vi "NEO Set Output.vi"(6 "Add Angle Offsets?":bool, 7 "Scaling":dbl, 8 "Arbitrary Feedforward":T1, 9 "Control Mode":T2, 10 "Setpoints":T1, 11 "Motors":cluster{"[0]":T3, "[1]":T3, "[2]":T3, "[3]":T3}) -> (3 "Setpoints Out":dbl[](array[numeric]))   [LabVIEW 2027]
uses:
  <vilib>/REV Custom Controls/REVSparkRefnum.ctl
  <vilib>/REV Custom Controls/Spark Output Control Type.ctl
  <vilib>/REVLibDriver/REVLibDriver.lvlib
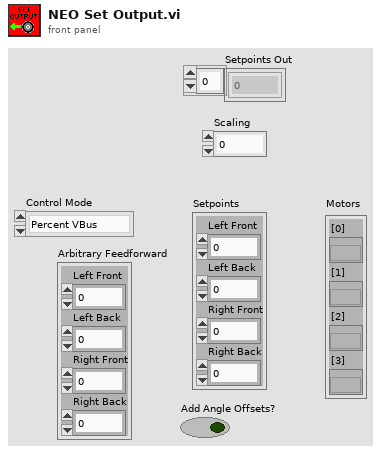
[diagram p1: front panel]
types:
  T1 = cluster{"Left Front":dbl, "Left Back":dbl, "Right Front":dbl, "Right Back":dbl}
  T2 = typedef "REVLibDriver.lvlib/Spark Output Control Type.ctl" = enum16{"Percent VBus", "Velocity", "Voltage", "Position", "Current", "MAXMotion Position", "MAXMotion Velocity"}
  T3 = typedef "REVLibDriver.lvlib/REVSparkRefnum.ctl" = refnum<k20>
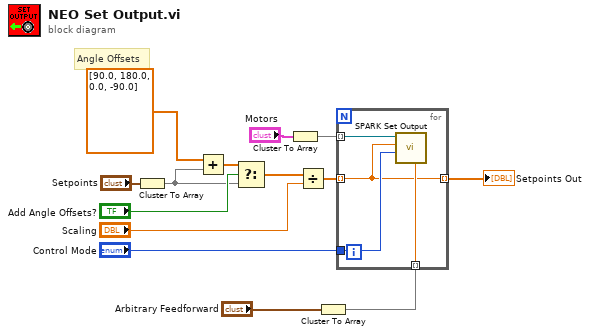
[diagram p0: block diagram]
diagram:
  # "Angle Offsets"
  n1 = Cluster To Array(cluster="Setpoints") -> (array=w7:dbl[])
  n2 = Add(x=dbl[] [90.0, 180.0, 0.0, -90.0] ("y"), y=w7) -> (x+y=w9:dbl[])
  n3 = Select(t=w9, s="Add Angle Offsets?", f=w7) -> (s? t:f=w3:dbl[])
  n4 = Cluster To Array(cluster="Motors") -> (array=w13:T3[])
  n5 = Divide(x=w3, y="Scaling") -> (x/y=w4:dbl[])
  n6 = Cluster To Array(cluster="Arbitrary Feedforward") -> (array=w5:dbl[])
  n7 = for {
    tunnel: w13 -> [w18] mode=indexing
    tunnel: w4 -> [w15] mode=indexing
    tunnel: "Control Mode" -> [w17]
    tunnel: w5 -> [w16] mode=indexing
    tunnel: [w15] -> w1 mode=indexing
    n8 = call <vilib>:"SPARK Set Output.vi"("Arbitrary Feed Forward (0)"=w16, "Control Mode"=w17, "Setpoint"=w15, "Spark refnum"=w18) -> ()  [unwired: 6 in, 2 out]
  }
  "Setpoints Out" <- w1
